vi "PID_Controller_Example.vi"() -> ()   [LabVIEW 2019]
uses:
  <vilib>/Rock Robotics/WPI/ThirdParty/JAS_Junk/TrajLib/Trajectory_Library.lvlib
  <vilib>/Rock Robotics/WPI/ThirdParty/JAS_Junk/TrajLib/LinearFilter_MovingAvg_Execute.vi
  <vilib>/Rock Robotics/WPI/ThirdParty/JAS_Junk/TrajLib/TypeDef/PID_CONTROLLER.ctl
  <vilib>/Rock Robotics/WPI/ThirdParty/JAS_Junk/TrajLib/TypeDef/PID_TUNING.ctl
panel:
  in  "Tab Control":T1(tab)
  in  "Enable Noise":bool=TRUE
  in  "Auto / Manual":bool=TRUE
  out "Dash Speed Demand":dbl format="%10.2f"
  in  "Desired Speed":dbl(slide)=-0.22222222222222499 scale=-50.0..50.0 scale format="%#.1f"
  out "Dash Speed Target":dbl format="%10.2f"
  out "DashRightMotorOutput":dbl format="%11.3f"
  out "DashRight Wheel Speed":dbl(knob)=-2.895988890827539e-05 scale=-60.0..60.0
  out "Right Wheel ErrorFilt":dbl format="%11.3f"
  out "Right Wheel SpeedFilt":dbl format="%10.2f"
  out "DashLeft Wheel Speed":dbl(knob)=-2.895988890827539e-05 scale=-60.0..60.0
  out "Left Wheel ErrorFilt":dbl format="%11.3f"
  out "DashLeftMotorOutput":dbl format="%11.3f"
  out "Left Wheel Speed Filt":dbl format="%10.2f"
  out "Left CO":dbl format="%13.3f"
  out "Right CO":dbl format="%13.3f"
  out "Duration":dbl format="%11.3f"
  out "Late":dbl format="%11.3f"
  out "SP, PV, CO Left":T2(graph)
  out "SP, PV, CO Right":T2(graph)
  in  "SetPoint Change Rate":dbl=80.0 min=1.0 max=9000.0 format="%14.4f"
  in  "PID Tuning Left":T3={"Kp"=0.4, "Ki"=2.0, "Kd"=0.0, "MaximumIntegral"=1.5, "MinimumIntegral"=-1.5, "IntegralZone"=9.9e+30}
  in  "PID Tuning Right":T3={"Kp"=0.4, "Ki"=2.0, "Kd"=0.0, "MaximumIntegral"=1.5, "MinimumIntegral"=-1.5, "IntegralZone"=9.9e+30}
  out "Left PID Data":T4={"Kp"=0.0, "Ki"=0.0, "Kd"=0.0, "Period"=0.0, "Max_Integral"=0.0, "Min_Integral"=0.0, "Max_Input"=0.0, "Min_Input"=0.0, "Continuous"=FALSE, "PositionError"=0.0, "VelocityError"=0.0, "PrevError"=0.0, "Total_Integral"=0.0, "PositionTolerance"=0.0, "VelocityTolerance"=0.0, "SetPoint"=0.0, "Kf"=0.0, "Prev_Deriv"=0.0, "Prev_Deriv 2"=0.0, "DerivativeFilter"=FALSE, "Min_Output"=-9.99e+35, "Max_Output"=9.9e+35, "Prev_F_P"=0.0, "Prev_F_P_2"=0.0, "AntiWindupActive"=FALSE, "Measurement"=0.0, "IntegralZone"=9.9e+30} {"IntegralZone" format="%16_6e"; "Measurement" format="%16_6e"; "Prev_F_P_2" format="%16_6e"; "Prev_F_P" format="%16_6e"; "Max_Output" format="%16_6e"; "Min_Output" format="%16_6e"; "Prev_Deriv 2" format="%16_6e"; "Prev_Deriv" format="%16_6e"; "Kf" format="%16_6e"; "SetPoint" format="%16_6e"; "VelocityTolerance" format="%16_6e"; "PositionTolerance" format="%16_6e"; "Total_Integral" format="%16_6e"; "PrevError" format="%16_6e"; "VelocityError" format="%16_6e"; "PositionError" format="%16_6e"; "Min_Input" format="%16_6e"; "Max_Input" format="%16_6e"; "Min_Integral" format="%16_6e"; "Max_Integral" format="%16_6e"; "Period" format="%16_6e"; "Kd" format="%16_6e"; "Ki" format="%16_6e"; "Kp" format="%16_6e"}
  out "Right PID Data":T4={"Kp"=0.0, "Ki"=0.0, "Kd"=0.0, "Period"=0.0, "Max_Integral"=0.0, "Min_Integral"=0.0, "Max_Input"=0.0, "Min_Input"=0.0, "Continuous"=FALSE, "PositionError"=0.0, "VelocityError"=0.0, "PrevError"=0.0, "Total_Integral"=0.0, "PositionTolerance"=0.0, "VelocityTolerance"=0.0, "SetPoint"=0.0, "Kf"=0.0, "Prev_Deriv"=0.0, "Prev_Deriv 2"=0.0, "DerivativeFilter"=FALSE, "Min_Output"=-9.99e+35, "Max_Output"=9.9e+35, "Prev_F_P"=0.0, "Prev_F_P_2"=0.0, "AntiWindupActive"=FALSE, "Measurement"=0.0, "IntegralZone"=9.9e+30} {"IntegralZone" format="%16_6e"; "Measurement" format="%16_6e"; "Prev_F_P_2" format="%16_6e"; "Prev_F_P" format="%16_6e"; "Max_Output" format="%16_6e"; "Min_Output" format="%16_6e"; "Prev_Deriv 2" format="%16_6e"; "Prev_Deriv" format="%16_6e"; "Kf" format="%16_6e"; "SetPoint" format="%16_6e"; "VelocityTolerance" format="%16_6e"; "PositionTolerance" format="%16_6e"; "Total_Integral" format="%16_6e"; "PrevError" format="%16_6e"; "VelocityError" format="%16_6e"; "PositionError" format="%16_6e"; "Min_Input" format="%16_6e"; "Max_Input" format="%16_6e"; "Min_Integral" format="%16_6e"; "Max_Integral" format="%16_6e"; "Period" format="%16_6e"; "Kd" format="%16_6e"; "Ki" format="%16_6e"; "Kp" format="%16_6e"}
  out "RightWheelSpeed":dbl
  out "LeftWheelSpeed":dbl
  out "RightMotorOutput":dbl
  out "LeftMotorOutput":dbl
  out "SpeedSetpoint":dbl
  in  "SpeedTarget":dbl
  in  "SpeedControlEnabled":bool
  # "PID Controller Example"
  # "This value shows the current speed of each wheel.  This is measured by an encoder.  The encoder measures\n speed by counting pulses of the wheel turning and dividing by the time interval.  Total distance change\nis also a result.  This value is called the \"Process Variable\"."
  # "Enter a desired speed and then press the Set Speed Target \nbutton.  This simulates the joystick input."
  # "FT/SEC"
  # "FT/SEC"
  # "FT/SEC"
  # "FT/SEC"
  # "The Speed Target is rate limited so not to make\nto drastic a change in the desired speed.  (This is\nwhat happens mechanically when pushing the gas\npedal of a real car.)"
  # "This error value shows the error between the current speed\nand the speed demand."
  # "FT/SEC"
  # "This example adds a \"Manual\" mode so that the still operates\nif the encoder fails."
  # "FT/SEC"
  # "FT/SEC"
  # "This value shows the current motor output demand.  This could also be a motor speed demand and \nanother closed loop controller would control the motor speed.  In this simple example this value is \nused to drive the simulated motor directly.  This motor demand is called the \"Control Output\"."
  # "Enables some simulated process noise"
  # "FT/SEC/SEC"
  # "These are the tuning parameters for the PID VI"
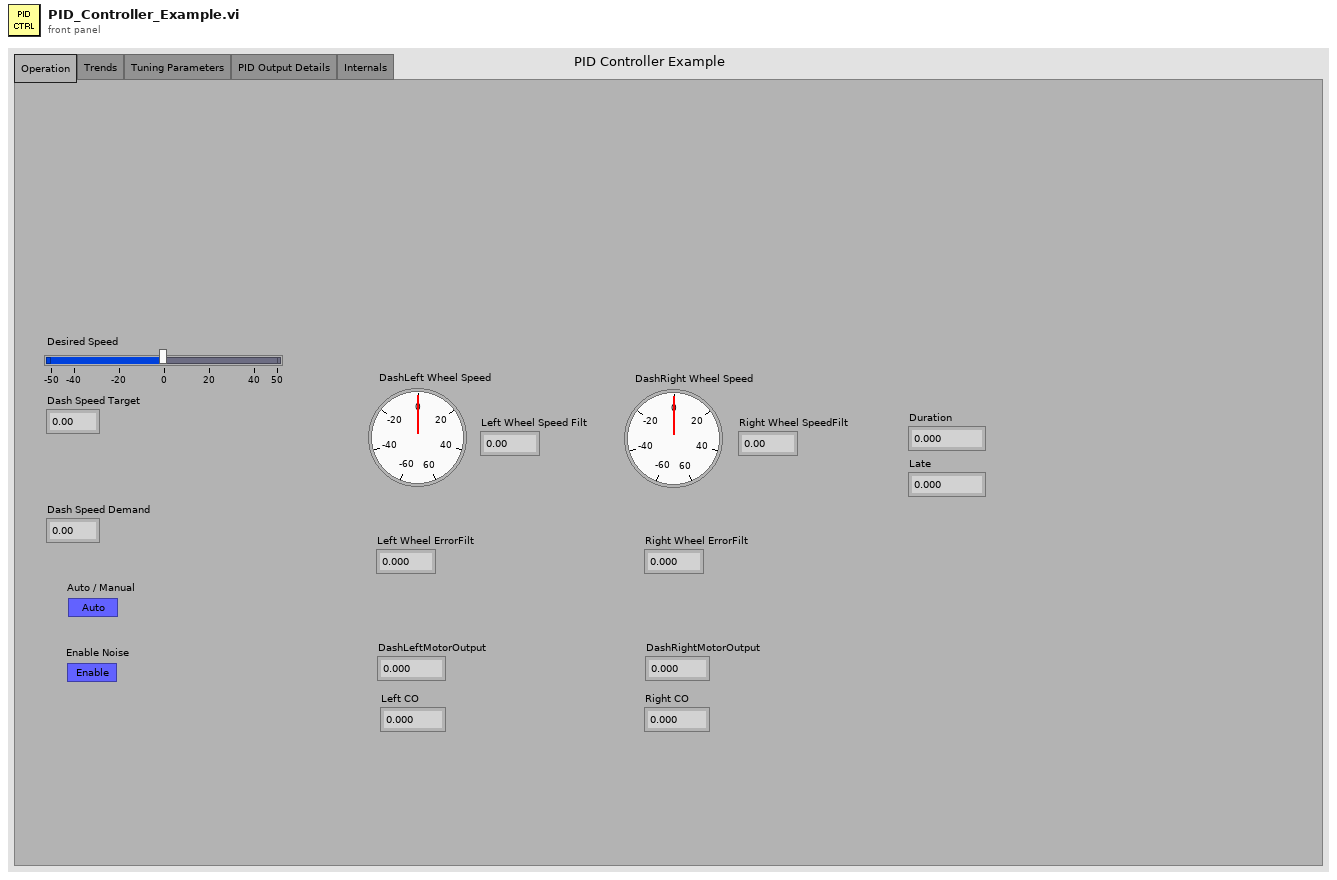
[diagram p1: front panel]
types:
  T1 = enum32{"Operation", "Trends", "Tuning Parameters", "PID Output Details", "Internals"}
  T2 = cluster{"MotorDemand":dbl, "CurrentSetpoint":dbl, "CurrentPosition":dbl}
  T3 = typedef "Trajectory_Library.lvlib/PID_TUNING.ctl" = cluster{"Kp":dbl, "Ki":dbl, "Kd":dbl, "MaximumIntegral":dbl, "MinimumIntegral":dbl, "IntegralZone":dbl}
  T4 = typedef "Trajectory_Library.lvlib/PID_CONTROLLER.ctl" = cluster{"Kp":dbl, "Ki":dbl, "Kd":dbl, "Period":dbl, "Max_Integral":dbl, "Min_Integral":dbl, "Max_Input":dbl, "Min_Input":dbl, "Continuous":bool, "PositionError":dbl, "VelocityError":dbl, "PrevError":dbl, "Total_Integral":dbl, "PositionTolerance":dbl, "VelocityTolerance":dbl, "SetPoint":dbl, "Kf":dbl, "Prev_Deriv":dbl, "Prev_Deriv 2":dbl, "DerivativeFilter":bool, "Min_Output":dbl, "Max_Output":dbl, "Prev_F_P":dbl, "Prev_F_P_2":dbl, "AntiWindupActive":bool, "Measurement":dbl, "IntegralZone":dbl}
  T5 = cluster{"LeftMotorOutput":dbl, "SpeedSetpoint":dbl, "LeftWheelSpeed":dbl}
  T6 = cluster{"RightMotorOutput":dbl, "SpeedSetpoint":dbl, "RightWheelSpeed":dbl}
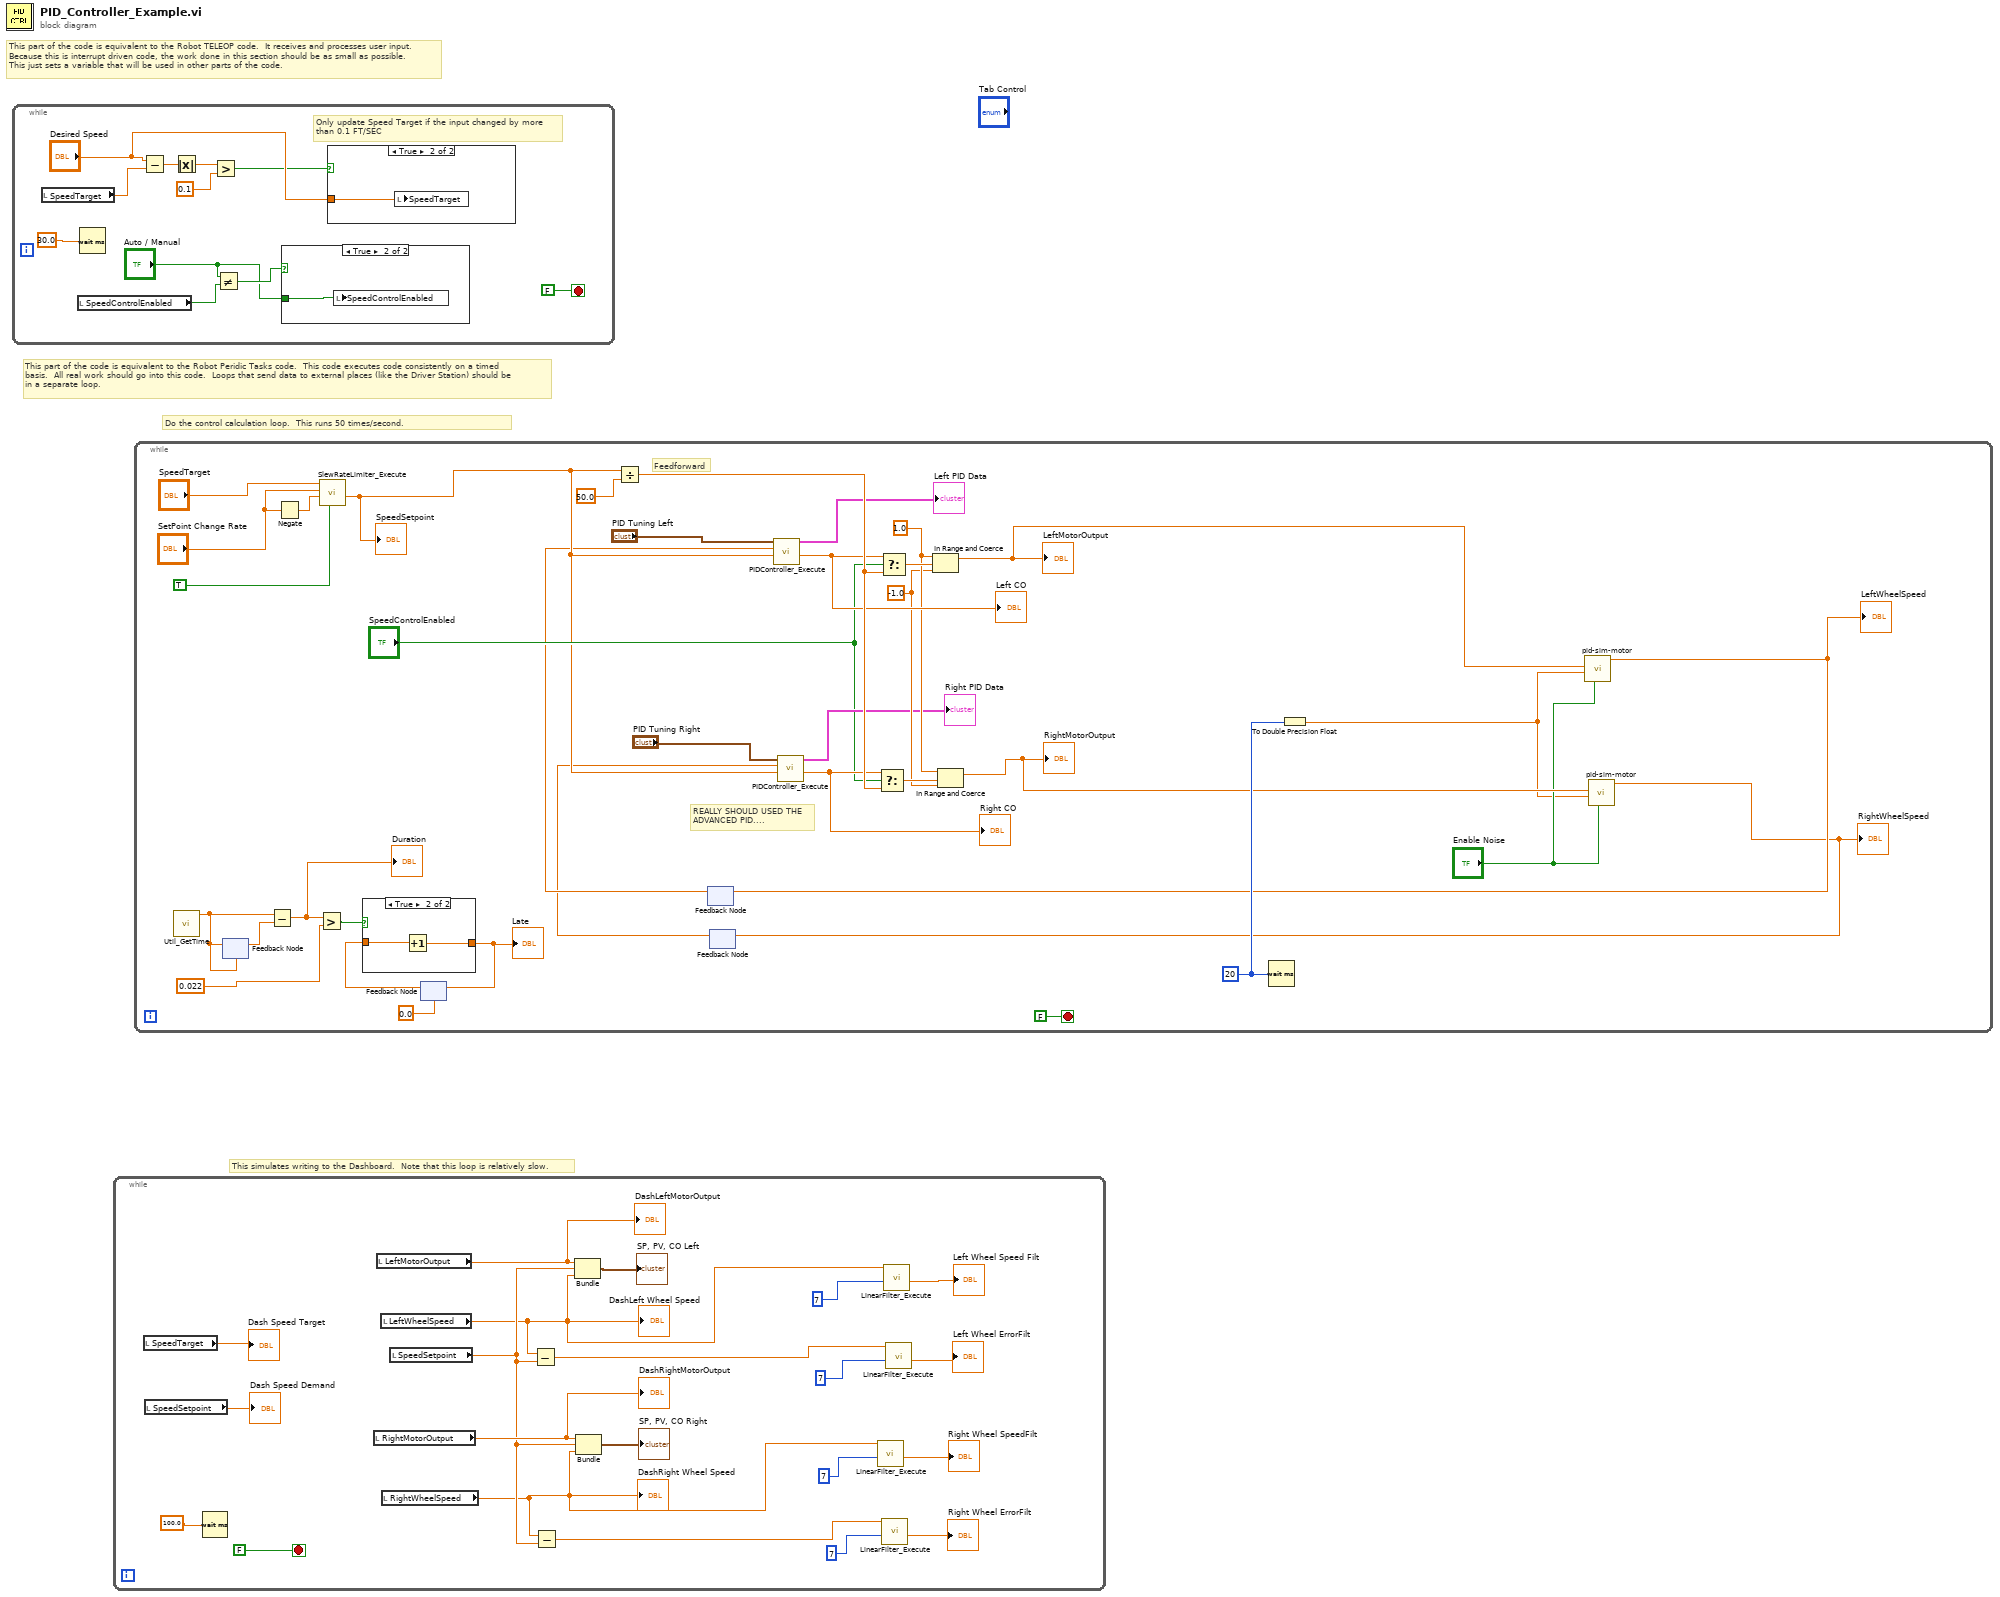
[diagram p0: block diagram]
diagram:
  # "This simulates writing to the Dashboard.  Note that this loop is relatively slow."
  # "Do the control calculation loop.  This runs 50 times/second."
  # "This part of the code is equivalent to the Robot Peridic Tasks code.  This code executes code consistently on a timed\nbasis.  All real work should go into this code.  Loops that send data to external places (like the Driver Station) should be \nin a separate loop."
  # "This part of the code is equivalent to the Robot TELEOP code.  It receives and processes user input.\nBecause this is interrupt driven code, the work done in this section should be as small as possible.\nThis just sets a variable that will be used in other parts of the code."
  n1 = while {
    stop <- FALSE stop-if-true
    # "Only update Speed Target if the input changed by more\nthan 0.1 FT/SEC"
    n2 = local read "SpeedTarget"() -> (w10:dbl)
    n3 = local read "SpeedControlEnabled"() -> (w2:bool)
    n4 = Wait (ms)(milliseconds to wait=30.0) -> ()  [unwired: 1 out]
    n5 = Subtract(x="Desired Speed", y=w10) -> (x-y=w9:dbl)
    n6 = Absolute Value(x=w9) -> (abs(x)=w8:dbl)
    n7 = Greater?(x=w8, y=0.1) -> (0:w5:bool)
    n8 = Not Equal?(x="Auto / Manual", y=w2) -> (x != y?=w3:bool)
    n9 = case shown="True" w3 {
      tunnel: "Auto / Manual" -> [_ w12]
      frame False {
      }
      frame True {
        n10 = local write "SpeedControlEnabled"(w12) -> ()
      }
    }
    n11 = case shown="True" w5 {
      tunnel: "Desired Speed" -> [_ w13]
      frame False {
      }
      frame True {
        n12 = local write "SpeedTarget"(w13) -> ()
      }
    }
  }
  n13 = while {
    stop <- FALSE stop-if-true
    n14 = local read "SpeedTarget"() -> (→"Dash Speed Target":dbl)
    n15 = local read "SpeedSetpoint"() -> (→"Dash Speed Demand":dbl)
    n16 = Wait (ms)(milliseconds to wait=100.0) -> ()  [unwired: 1 out]
    n17 = local read "RightMotorOutput"() -> (w30:dbl)
    "DashRightMotorOutput" <- w30
    n18 = local read "LeftMotorOutput"() -> (w27:dbl)
    "DashLeftMotorOutput" <- w27
    n19 = local read "LeftWheelSpeed"() -> (w24:dbl)
    "DashLeft Wheel Speed" <- w24
    n20 = local read "RightWheelSpeed"() -> (w17:dbl)
    "DashRight Wheel Speed" <- w17
    n21 = local read "SpeedSetpoint"() -> (w26:dbl)
    n22 = Subtract(x=w24, y=w26) -> (x-y=w21:dbl)
    n23 = Subtract(x=w17, y=w26) -> (x-y=w14:dbl)
    n24 = Bundle("LeftMotorOutput"=w27, "SpeedSetpoint"=w26, "LeftWheelSpeed"=w24) -> (→"SP, PV, CO Left":T5)  [unwired: 1 in]
    n25 = Bundle("RightMotorOutput"=w30, "SpeedSetpoint"=w26, "RightWheelSpeed"=w17) -> (→"SP, PV, CO Right":T6)  [unwired: 1 in]
    n26 = call-poly <vilib>:"LinearFilter_Execute.vi"("Samples"=7, "Input"=w17) -> ("Output"=→"Right Wheel SpeedFilt":dbl)  [unwired: 9 in]
    n27 = call-poly <vilib>:"LinearFilter_Execute.vi"("Samples"=7, "Input"=w14) -> ("Output"=→"Right Wheel ErrorFilt":dbl)  [unwired: 9 in]
    n28 = call-poly <vilib>:"LinearFilter_Execute.vi"("Samples"=7, "Input"=w24) -> ("Output"=→"Left Wheel Speed Filt":dbl)  [unwired: 9 in]
    n29 = call-poly <vilib>:"LinearFilter_Execute.vi"("Samples"=7, "Input"=w21) -> ("Output"=→"Left Wheel ErrorFilt":dbl)  [unwired: 9 in]
  }
  n30 = while {
    stop <- FALSE stop-if-true
    w63 = -1.0 ("lower limit")
    w64 = 1.0 ("upper limit")
    w48 = u32 20 ("milliseconds to wait")
    # "REALLY SHOULD USED THE\nADVANCED PID...."
    # "Feedforward"
    n31 = call <vilib>:"Util_GetTime.vi"() -> ("FPGA_Time_Seconds"=w57:dbl)  [unwired: 9 in, 2 out]
    n32 = feedback #1(w57) -> (w56:dbl)
    n33 = feedback-in #1(w57) -> ()
    n34 = Subtract(x=w57, y=w56) -> (x-y=w54:dbl)
    "Duration" <- w54
    n35 = Negate(x="SetPoint Change Rate") -> (-x=w43:dbl)
    n36 = Greater?(x=w54, y=0.022) -> (0:w55:bool)
    n37 = call <vilib>:"SlewRateLimiter_Execute.vi"("Enable"=TRUE, "NegativeRate"=w43, "PositiveRate"="SetPoint Change Rate", "Input"="SpeedTarget") -> ("Output"=w49:dbl)  [unwired: 6 in, 1 out]
    "SpeedSetpoint" <- w49
    n38 = feedback #2(0.0) -> (w58:dbl)
    n39 = case shown="True" w55 {
      tunnel: [w71 w73] -> w59
      tunnel: w58 -> [w71 w72]
      frame False {
      }
      frame True {
        n40 = Increment(x=w72) -> (x+1=w73:dbl)
      }
    }
    "Late" <- w59
    n41 = feedback-in #2(w59) -> ()
    n42 = Divide(x=w49, y=50.0) -> (x/y=w69:dbl)
    n43 = feedback #3() -> (w47:dbl)  [unwired: 1 in]
    n44 = feedback #4() -> (w46:dbl)  [unwired: 1 in]
    n45 = call <vilib>:"PIDController_Execute.vi"("SP-SetPoint"=w49, "PV-Measurement"=w47, "PID Tuning"="PID Tuning Left") -> ("CO-ControlOutput"=w67:dbl, "out PID_CONTROLLER"=→"Left PID Data":T4)  [unwired: 6 in, 1 out]
    "Left CO" <- w67
    n46 = call <vilib>:"PIDController_Execute.vi"("SP-SetPoint"=w49, "PV-Measurement"=w46, "PID Tuning"="PID Tuning Right") -> ("CO-ControlOutput"=w60:dbl, "out PID_CONTROLLER"=→"Right PID Data":T4)  [unwired: 6 in, 1 out]
    "Right CO" <- w60
    n47 = Select(t=w60, s="SpeedControlEnabled", f=w69) -> (s? t:f=w65:dbl)
    n48 = Select(t=w67, s="SpeedControlEnabled", f=w69) -> (s? t:f=w66:dbl)
    n49 = In Range and Coerce(upper limit=w64, x=w66, lower limit=w63) -> (coerced(x)=w42:dbl)  [unwired: 1 out]
    "LeftMotorOutput" <- w42
    n50 = In Range and Coerce(upper limit=w64, x=w65, lower limit=w63) -> (coerced(x)=w40:dbl)  [unwired: 1 out]
    "RightMotorOutput" <- w40
    n51 = Wait (ms)(milliseconds to wait=w48) -> ()  [unwired: 1 out]
    n52 = To Double Precision Float(number=w48) -> (double precision float=w37:dbl)
    n53 = call "pid-sim-motor.vi"("Use Noise"="Enable Noise", "Cycle Time"=w37, "CO-ControlOutput"=w42) -> ("Motor Speed"=w41:dbl)  [unwired: 8 in]
    "LeftWheelSpeed" <- w41
    n54 = feedback-in #3(w41) -> ()
    n55 = call "pid-sim-motor.vi"("Use Noise"="Enable Noise", "Cycle Time"=w37, "CO-ControlOutput"=w40) -> ("Motor Speed"=w39:dbl)  [unwired: 8 in]
    "RightWheelSpeed" <- w39
    n56 = feedback-in #4(w39) -> ()
  }
